vi "Test Incoming Measurement Error.vi"() -> (0 "error out":errorcluster)   [LabVIEW 2026]
doc: "BUF-003: the full incoming error cluster must survive the Standard Measurement buffered read."
uses:
  source/plugins/measurements/Standard Measurement Plugin/Standard Measurement.lvclass
  <vilib>/addons/_JKI Toolkits/Caraya/classes/Test/Test.lvclass
  <vilib>/addons/_JKI Toolkits/Caraya/classes/Assert/Assert.lvclass
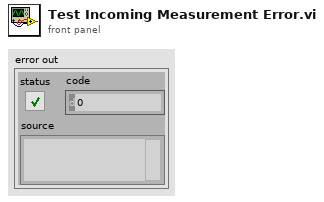
[diagram p1: front panel]
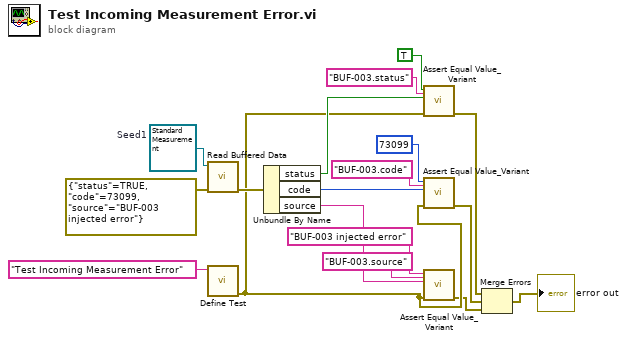
[diagram p0: block diagram]
diagram:
  w16 = refnum<class "Standard Measurement.lvclass"> refnum  # Seed1
  n1 = call "Read Buffered Data.vi"("error in (no error)"=errorcluster {"status"=TRUE, "code"=73099, "source"="BUF-003 injected error"}, "Standard Measurement in"=w16) -> ("error out"=w15:errorcluster)  [unwired: 8 in, 1 out]
  n2 = call <vilib>:"Define Test.vi"("Label (VI Title)"="Test Incoming Measurement Error") -> ("error out"=w8:errorcluster)  [unwired: 9 in, 1 out]
  n3 = Unbundle By Name(w15) -> ("status"=w13:bool, "code"=w10:i32, "source"=w6:string)
  n4 = call <vilib>:"Assert Equal Value_Variant.vi"("Label"="BUF-003.status", "error in (no error)"=w8, "Actual"=w13, "Expected"=TRUE) -> ("error out"=w4:errorcluster)  [unwired: 6 in, 1 out]
  n5 = call <vilib>:"Assert Equal Value_Variant.vi"("Label"="BUF-003.code", "error in (no error)"=w8, "Actual"=w10, "Expected"=73099) -> ("error out"=w3:errorcluster)  [unwired: 6 in, 1 out]
  n6 = call <vilib>:"Assert Equal Value_Variant.vi"("Label"="BUF-003.source", "error in (no error)"=w8, "Actual"=w6, "Expected"="BUF-003 injected error") -> ("error out"=w2:errorcluster)  [unwired: 6 in, 1 out]
  n7 = Merge Errors(w4, w3, w2) -> (→"error out":errorcluster)
